vi "RDC-Lin-Find_probe_char.vi"(10 "Open Probe reading":T1={"Frequency"=array[2001 elements], "Reflection'"=array[2001 elements], "Reflection''"=array[2001 elements], "Permativity'"=array[2001 elements], "Permativity''"=array[2001 elements], "Conductivity"=array[2001 elements], "Loss Tangent"=array[2001 elements], "Resistance"=[], "Reactance"=[]}, 11 "Short Probe reading":T1={"Frequency"=array[2001 elements], "Reflection'"=array[2001 elements], "Reflection''"=array[2001 elements], "Permativity'"=array[2001 elements], "Permativity''"=array[2001 elements], "Conductivity"=array[2001 elements], "Loss Tangent"=array[2001 elements], "Resistance"=[], "Reactance"=[]}) -> (2 "C0":dbl format="%#_6p", 3 "Tau":dbl format="%#_6p")   [LabVIEW 2020, in "RDC-Reflection_Data_Computation.lvlib"]
doc: "Finds the probe characteristics C0 and Tau from an open-probe and a short-probe Common Format cluster."
uses:
  RDC-Reflection_Data_Computation.lvlib
  Reflector/RFH-common_data_format.ctl
  Reflector/RFH-Reflection_File_Handler.lvlib
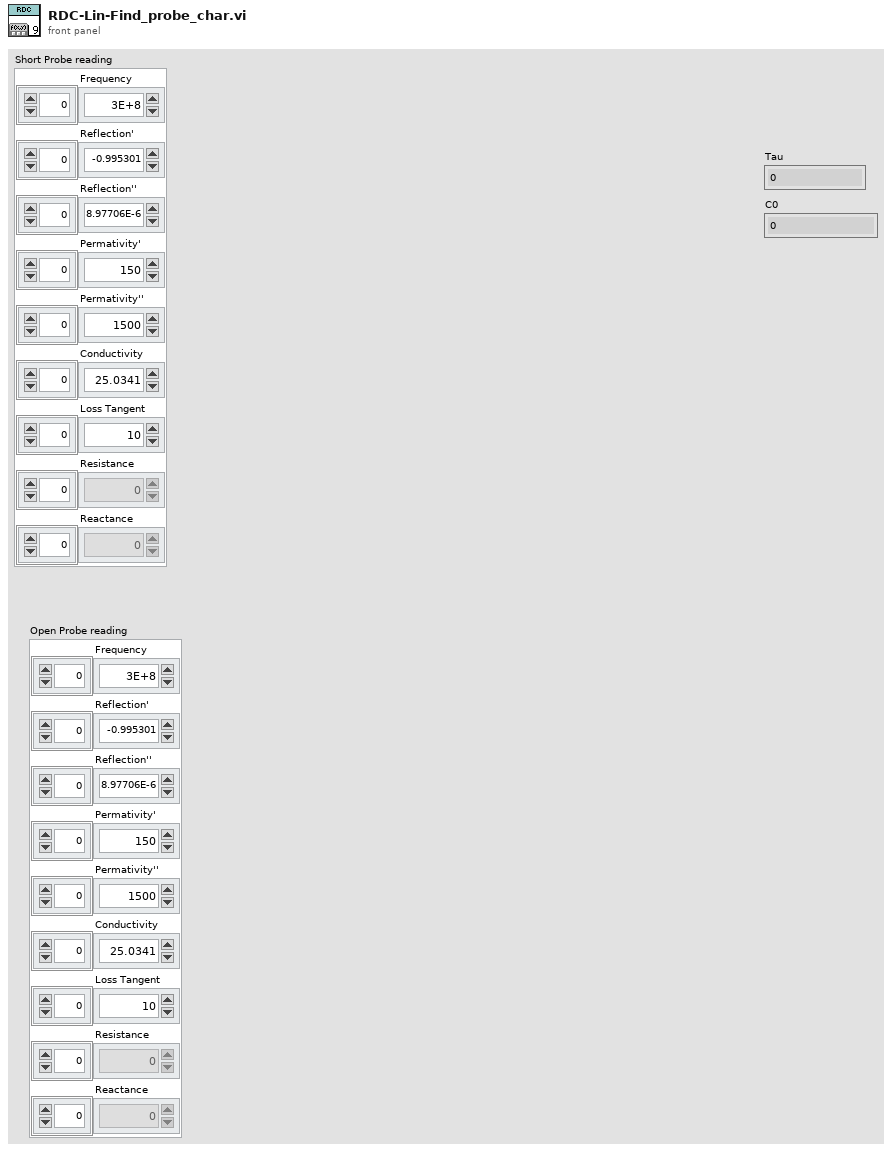
[diagram p1: front panel]
types:
  T1 = typedef "RFH-Reflection_File_Handler.lvlib/RFH-common_data_format.ctl" = cluster{"Frequency":dbl[], "Reflection'":dbl[], "Reflection''":dbl[], "Permativity'":dbl[], "Permativity''":dbl[], "Conductivity":dbl[], "Loss Tangent":dbl[], "Resistance":dbl[], "Reactance":dbl[]}
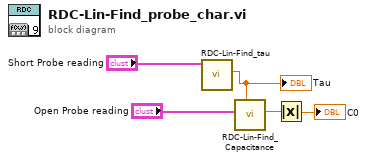
[diagram p0: block diagram]
diagram:
  n1 = call "RDC-Lin-Find_tau.vi"("Short Probe reading"="Short Probe reading") -> ("Tau"=w2:dbl)  [unwired: 9 in, 1 out]
  "Tau" <- w2
  n2 = call "RDC-Lin-Find_Capacitance.vi"("Tau"=w2, "Open Probe reading"="Open Probe reading") -> ("C0"=w5:dbl)  [unwired: 9 in]
  n3 = Absolute Value(x=w5) -> (abs(x)=→"C0":dbl)
